vi "SignalAndSpectrum.vi"(7 "LabVIEW Web Service Request":refnum<class "Web Request.lvclass">) -> ()   [LabVIEW 2016]
uses:
  <vilib>/wsapi/Web Request.lvclass
  <vilib>/Analysis/2dsp.llb/Power Spectrum (DBL).vi
  <vilib>/Analysis/NI_AALBase.lvlib
  <vilib>/Analysis/NI_AALPro.lvlib
panel:
  # "Use the Web Service Request input terminal to call the VIs on the Web Services palette. Do not remove it from the connector pane unless you don't need access to the palette."
  # "Each additional control wired to the connector pane will be available as an input in the URL. To include an indicator in terminal-mode output (the default setting), it must also be wired to the connector pane."
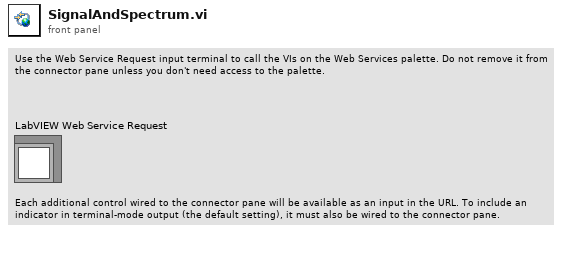
[diagram p1: front panel]
types:
  T1 = cluster{"Amplitude":dbl, "Samples":i32, "Frequency":dbl, "Noise%":dbl}
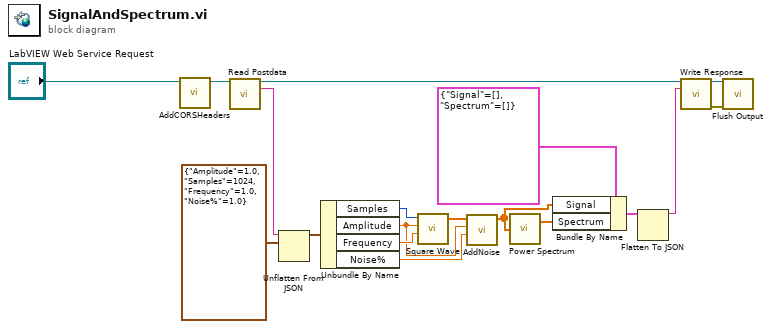
[diagram p0: block diagram]
diagram:
  n1 = call "AddCORSHeaders.vi"("Web Request in"="LabVIEW Web Service Request") -> ("Web Request out"=w11:refnum<class "Web Request.lvclass">)  [unwired: 10 in]
  n2 = call <vilib>:"Read Postdata.vi"("LabVIEW Web Service Request"=w11) -> ("LabVIEW Web Service Request out"=w10:refnum<class "Web Request.lvclass">, "postdata"=w18:string)  [unwired: 12 in, 1 out]
  n3 = Unflatten From JSON(JSON string=w18, type and defaults=T1 {"Amplitude"=1.0, "Samples"=1024, "Frequency"=1.0, "Noise%"=1.0}) -> (value=w16:T1)  [unwired: 5 in, 1 out]
  n4 = Unbundle By Name(w16) -> ("Samples"=w8:i32, "Amplitude"=w5:dbl, "Frequency"=w7:dbl, "Noise%"=w6:dbl)
  n5 = call <vilib>:"Square Wave.vi"("samples"=w8, "amplitude"=w5, "frequency"=w7) -> ("square wave"=w14:dbl[])  [unwired: 3 in, 2 out]
  n6 = call "AddNoise.vi"("Level (%)"=w6, "Signal Amplitude"=w5, "Signal In"=w14) -> ("Signal Out"=w13:dbl[])  [unwired: 8 in]
  n7 = call-poly <vilib>:"Power Spectrum.vi"("X"=w13) -> ("Power Spectrum"=w15:dbl[])  [unwired: 1 out]
  n8 = Bundle By Name(cluster=cluster{"Signal":dbl[], "Spectrum":dbl[]} {"Signal"=[], "Spectrum"=[]}, "Signal"=w13, "Spectrum"=w15) -> (w3:cluster{"Signal":dbl[], "Spectrum":dbl[]})
  n9 = Flatten To JSON(anything=w3) -> (JSON string=w9:string)  [unwired: 2 in, 1 out]
  n10 = call <vilib>:"Write Response.vi"("LabVIEW Web Service Request"=w10, "response string"=w9) -> ("LabVIEW Web Service Request out"=w1:refnum<class "Web Request.lvclass">, "error out"=w2:errorcluster)  [unwired: 12 in]
  n11 = call <vilib>:"Flush Output.vi"("LabVIEW Web Service Request"=w1, "error in (no error)"=w2) -> ()  [unwired: 12 in, 2 out]
